vi "Inspect Basic Flags on Structure Tunnels.vi"(8 "error in (no error)":errorcluster, 11 "Struct Refnum":refnum<vi>) -> (0 "error out":errorcluster, 3 "reference out":refnum<vi>)   [LabVIEW 2012, in "Scripting Tools.lvlib"]
uses:
  Scripting Tools.lvlib
  <vilib>/Utility/miscctls.llb/LVPositionTypeDef.ctl
panel:
  out "Array":T2(array[cluster])
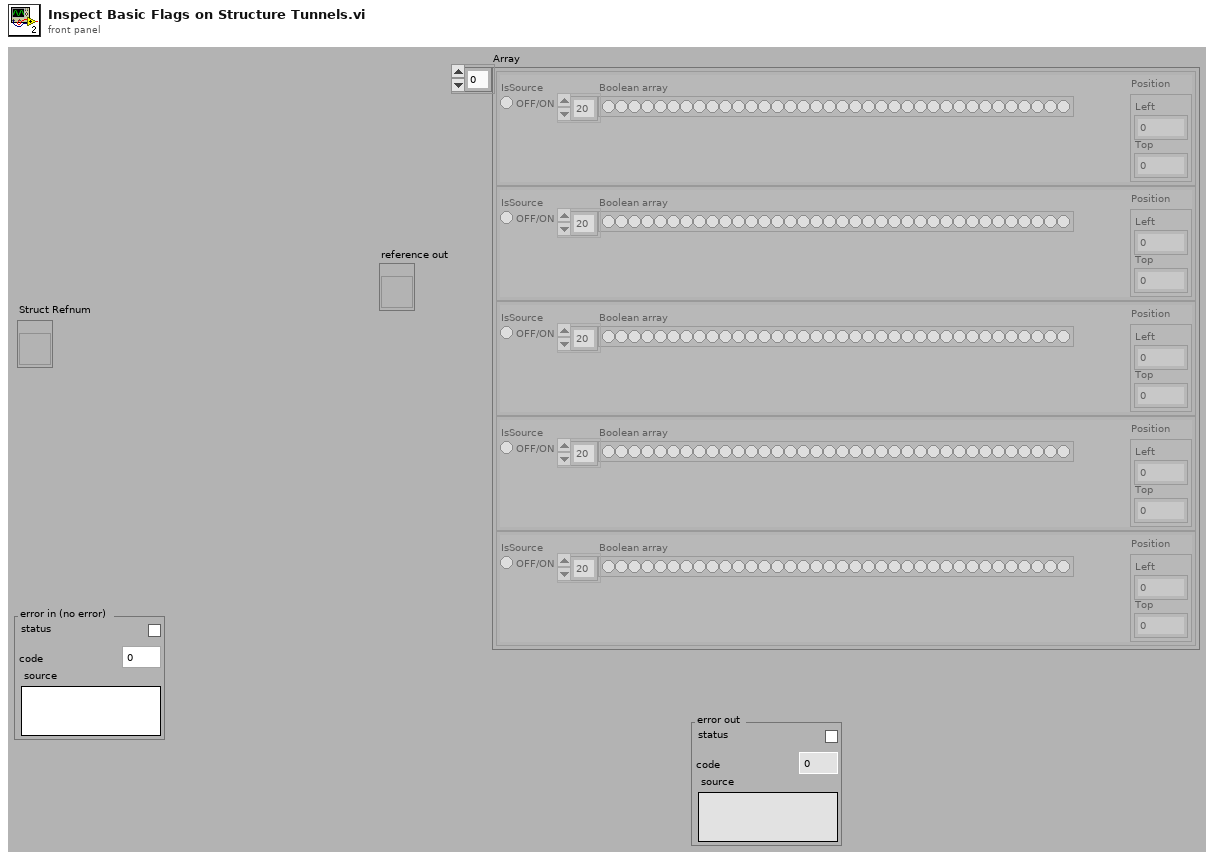
[diagram p1: front panel]
types:
  T1 = typedef "LVPositionTypeDef.ctl" = cluster{"Left":i32, "Top":i32}
  T2 = cluster{"IsSource":bool, "Boolean array":bool[], "Position":T1}[]
  T3 = cluster{"IsSource":bool, "Boolean array":bool[], "Position":T1}
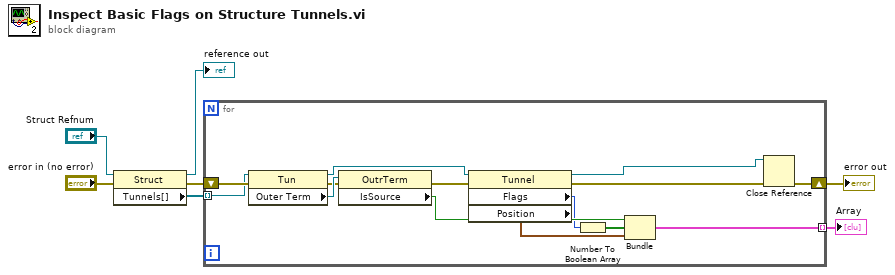
[diagram p0: block diagram]
diagram:
  n1 = property class="Struct"(reference="Struct Refnum", error in="error in (no error)") -> (reference out=→"reference out":refnum<vi>, error out=w4:errorcluster, "Tunnels[]"=w5:refnum<vi>[])
  n2 = for {
    tunnel: w5 -> [w20] mode=indexing
    shift-right: [w14] -> w2
    shift-left: w4 -> [w21]
    tunnel: [w8] -> w1 mode=indexing
    n3 = property class="Tun"(reference=w20, error in=w21) -> (reference out=w17:refnum<vi>, error out=w18:errorcluster, "Outer Term"=w19:refnum<vi>)
    n4 = property class="OutrTerm"(reference=w19, error in=w18) -> (error out=w16:errorcluster, "IsSource"=w12:bool)  [unwired: 1 out]
    n5 = property class="Tunnel"(reference=w17, error in=w16) -> (reference out=w13:refnum<vi>, error out=w15:errorcluster, "Flags"=w11:u32, "Position"=w10:T1)
    n6 = Number To Boolean Array(number=w11) -> (Boolean array=w9:bool[])
    n7 = Bundle("IsSource"=w12, "Boolean array"=w9, "Position"=w10) -> (w8:T3)  [unwired: 1 out]
    n8 = Close Reference(reference=w13, error in (no error)=w15) -> (error out=w14:errorcluster)
  }
  "error out" <- w2
  "Array" <- w1
